vi "串口读写 - 步进电机 - MO1.vi"(7 "寄存器地址":u8, 8 "错误输入（无错误）":errorcluster, 9 "写/读":bool, 10 "写入数据":i32, 11 "VISA输入":refnum<visa-resource-name>) -> (0 "错误输出":errorcluster, 1 "读取设备(n)":i32, 2 "报错":bool, 3 "VISA输出":refnum<visa-resource-name>)   [LabVIEW 2026, in "UI-步进.lvlib"]
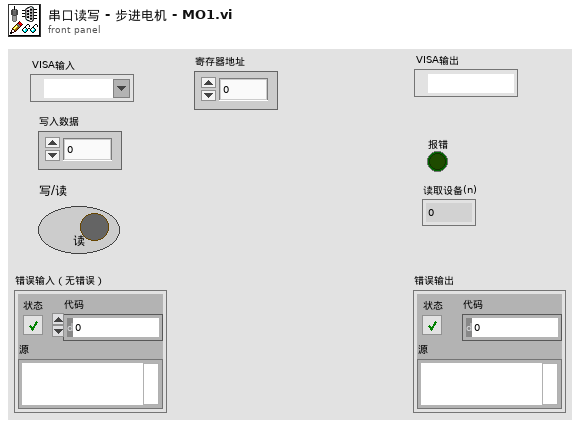
[diagram p1: front panel]
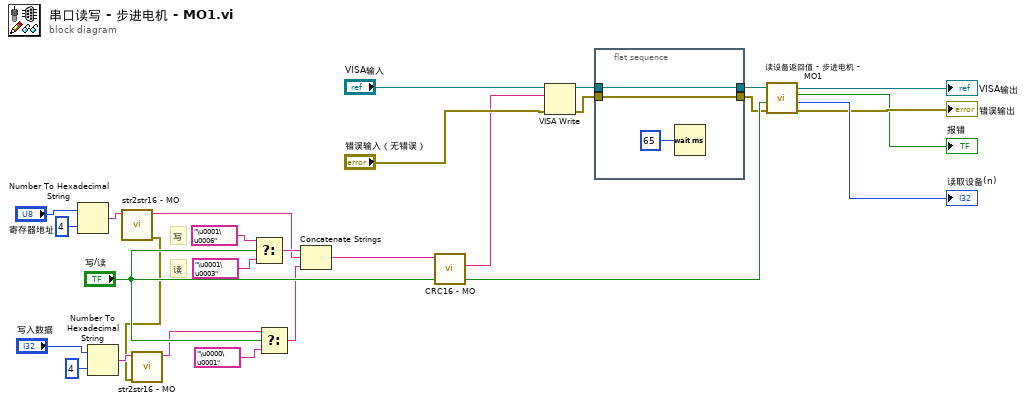
[diagram p0: block diagram]
diagram:
  # "写"
  # "读"
  n1 = Number To Hexadecimal String(1:i16 4 ("宽度(-)"), 2:"寄存器地址") -> (0:w12:string)
  n2 = Number To Hexadecimal String(1:i16 4 ("宽度(-)"), 2:"写入数据") -> (0:w16:string)
  n3 = call "str2str16 - MO.vi"("字符串"=w12) -> ("错误输出"=w1:errorcluster, "string"=w10:string)  [unwired: 9 in]
  n4 = call "str2str16 - MO.vi"("错误输入"=w1, "字符串"=w16) -> ("string"=w14:string)  [unwired: 8 in, 1 out]
  n5 = Select(t="\u0001\u0006" ("Command"), s="写/读", f="\u0001\u0003" ("Command")) -> (s? t:f=w23:string)
  n6 = Select(t=w14, s="写/读", f="\u0000\u0001" ("Command")) -> (s? t:f=w20:string)
  n7 = Concatenate Strings(w23, w10, w20) -> (w19:string)
  n8 = call "CRC16 - MO.vi"("要校验的字符串（十六进制显示）"=w19) -> ("连接的字符串(16进制)"=w18:string)  [unwired: 9 in, 1 out]
  n9 = VISA Write(VISA resource name="VISA输入", write buffer=w18, error in (no error)="错误输入（无错误）") -> (VISA resource name out=w5:refnum<visa-resource-name>, error out=w4:errorcluster)  [unwired: 1 out]
  n10 = flat-sequence {
    tunnel: [w30] -> w6
    tunnel: w5 -> [w30]
    tunnel: w4 -> [w29]
    tunnel: [w29] -> w3
    frame #0 {
      n11 = Wait (ms)(milliseconds to wait=u32 65 ("等待时间（毫秒）")) -> ()  [unwired: 1 out]
    }
  }
  n12 = call "读设备返回值 - 步进电机 - MO1.vi"("错误输入（无错误）"=w3, "写/读"="写/读", "VISA引用句柄输入"=w6) -> ("错误输出"=→"错误输出":errorcluster, "读取设备(n)"=→"读取设备(n)":i32, "报错"=→"报错":bool, "VISA引用句柄输出"=→"VISA输出":refnum<visa-resource-name>)  [unwired: 5 in]
